vi "ADC.vi"(0 "Input Voltage":dbl, 5 "Reference Voltage":dbl, 7 "Resolution":u16, 11 "Error In":errorcluster) -> (4 "Code":i32, 6 "LSB":dbl, 15 "Error Out":errorcluster)   [LabVIEW 2026, in "Core.lvlib"]
doc: "Simulates ADC conversion by converting an input voltage into a digital output code based on the configured resolution and reference voltage."
uses:
  Core.lvlib
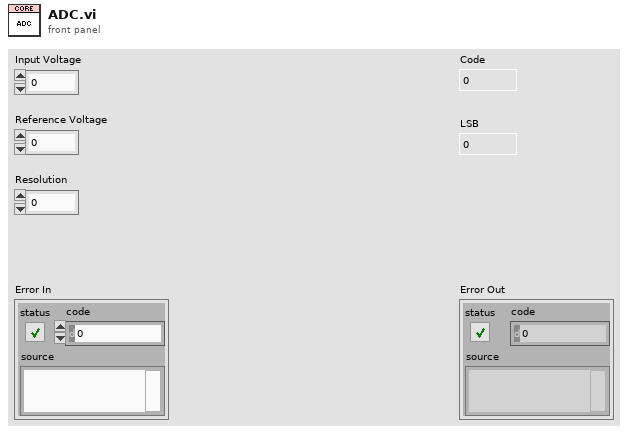
[diagram p1: front panel]
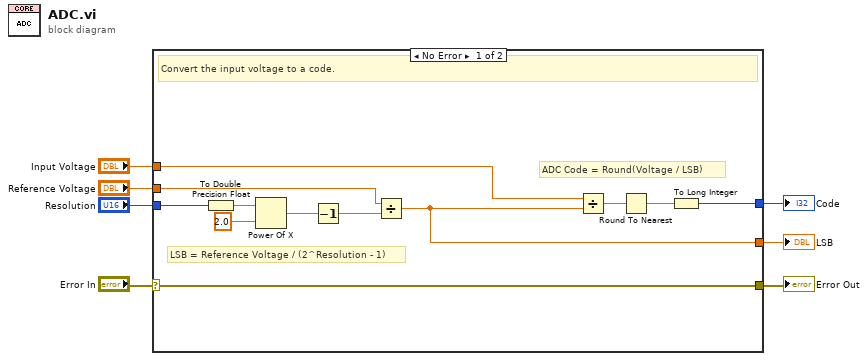
[diagram p0: block diagram]
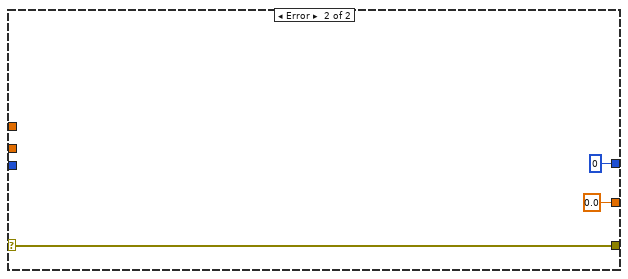
[diagram p2: hidden frame]
diagram:
  n1 = case shown="No Error" "Error In" {
    selector: "Error In" -> [w10 w22]
    tunnel: "Resolution" -> [w18 _]
    tunnel: "Reference Voltage" -> [w14 _]
    tunnel: "Input Voltage" -> [w13 _]
    tunnel: [w10 w22] -> w4
    tunnel: [w9 0] -> w2
    tunnel: [w8 0.0] -> w1
    frame No Error {
      # "ADC Code = Round(Voltage / LSB)"
      # "LSB = Reference Voltage / (2^Resolution - 1)"
      # "Convert the input voltage to a code."
      n2 = To Double Precision Float(number=w18) -> (double precision float=w17:dbl)
      n3 = Power Of X(1:2.0 ("x"), 2:w17) -> (0:w16:dbl)
      n4 = Decrement(x=w16) -> (x-1=w15:dbl)
      n5 = Divide(x=w14, y=w15) -> (x/y=w8:dbl)
      n6 = Divide(x=w13, y=w8) -> (x/y=w12:dbl)
      n7 = Round To Nearest(number=w12) -> (nearest integer value=w11:dbl)
      n8 = To Long Integer(number=w11) -> (32bit integer=w9:i32)
    }
    frame Error {
    }
  }
  "Error Out" <- w4
  "Code" <- w2
  "LSB" <- w1
